vi "Rename lvlib.vi"(8 "error in":errorcluster, 9 "New Name":string, 10 "Library":string, 11 "Project Manager in":refnum<class "Project Manager.lvclass">) -> (0 "error out":errorcluster, 3 "Project Manager out":refnum<class "Project Manager.lvclass">)   [LabVIEW 2026, in "Project Manager.lvclass"]
doc: "Rename a library (.lvlib) to the provided new name. This VI renames both the project item and the file."
uses:
  Project Manager.lvclass
  Project Manager.lvclass/Project Manager.ctl
  Interfaces/ILogger/ILogger Messages/Log Msg/Log Msg.lvclass/Log Msg.ctl
  <vilib>/ActorFramework/Message Enqueuer/Message Enqueuer.lvclass/Message Enqueuer.ctl
  <vilib>/ActorFramework/Message Enqueuer/Enqueue.vi
  Interfaces/ILogger/ILogger Messages/Log Msg/Log Msg.lvclass
  <userlib>/_OpenG.lib/file/file.llb/Convert File Extension (Path)__ogtk.vi
  <vilib>/ActorFramework/Message Priority Queue/Priority Enqueue.vi
  <userlib>/_OpenG.lib/file/file.llb/openg_file.lvlib
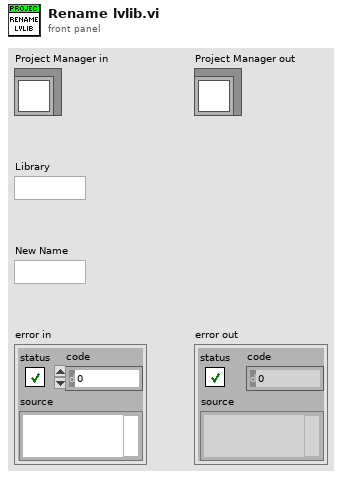
[diagram p1: front panel]
types:
  T1 = typedef "Log Entry--cluster.ctl" = cluster{"Time":timestamp, "Message":string}
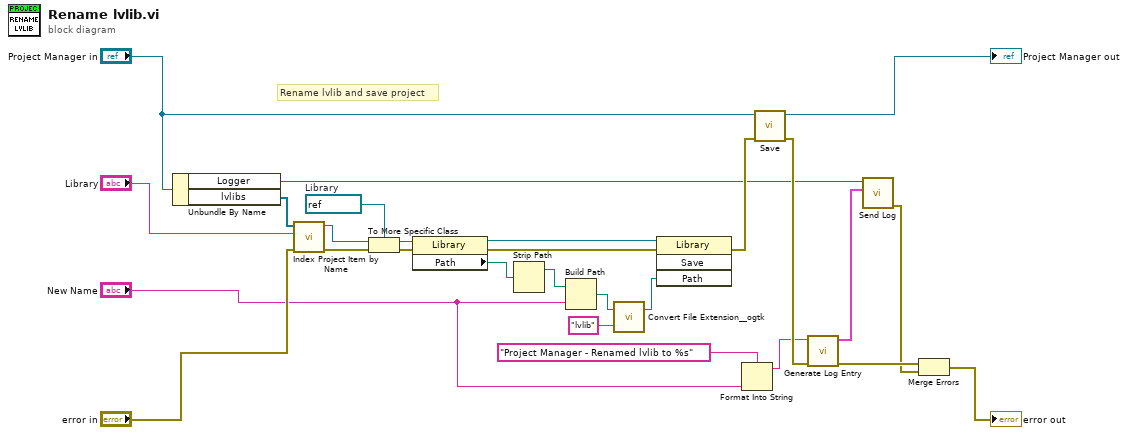
[diagram p0: block diagram]
diagram:
  w7 = refnum<vi> refnum  # Library
  # "Rename lvlib and save project"
  n1 = Unbundle By Name("Project Manager in") -> ("Logger"=w5:refnum<class "Message Enqueuer.lvclass">, "lvlibs"=w14:refnum<vi>[])
  n2 = call "Index Project Item by Name.vi"("error in"="error in", "Name"="Library", "Project Items"=w14) -> ("error out"=w24:errorcluster, "Project Item"=w8:refnum<vi>)  [unwired: 7 in]
  n3 = To More Specific Class(target class=w7, reference=w8, error in=w24) -> (specific class reference=w6:refnum<vi>, error out=w23:errorcluster)
  n4 = property class="Library"(reference=w6, error in=w23) -> (reference out=w12:refnum<vi>, error out=w25:errorcluster, "Path"=w11:path)
  n5 = Strip Path(path=w11) -> (stripped path=w10:path)  [unwired: 1 out]
  n6 = Build Path(base path=w10, name or relative path="New Name") -> (appended path=w9:path)
  n7 = call-poly <userlib>:"Convert File Extension__ogtk.vi"("new ending (none)"="lvlib", "file name"=w9) -> ("new filename"=w17:path)  [unwired: 1 out]
  n8 = invoke class="Library" method="Save"(reference=w12, error in=w25, "Path"=w17) -> (error out=w27:errorcluster)  [unwired: 1 in, 3 out]
  n9 = Format Into String(format string="Project Manager - Renamed lvlib to %s", "New Name") -> (resulting string=w1:string)  [unwired: 2 in, 1 out]
  n10 = call-dynamic "Save.vi"("error in"=w27, "Project Manager in"="Project Manager in") -> ("error out"=w22:errorcluster, "Project Manager out"=→"Project Manager out":refnum<class "Project Manager.lvclass">)  [unwired: 8 in]
  n11 = call "Generate Log Entry.vi"("error in"=w22, "Message"=w1) -> ("error out"=w21:errorcluster, "Log Entry"=w4:T1)  [unwired: 8 in]
  n12 = call "Send Log.vi"("Log Entry"=w4, "Message Enqueuer"=w5) -> ("error out"=w19:errorcluster)  [unwired: 8 in, 1 out]
  n13 = Merge Errors(w21, w19) -> (→"error out":errorcluster)
